vi "Dispose.vi"(8 "error in (no error)":errorcluster, 11 "ChangeNotifier in":refnum<class "ChangeNotifier.lvclass">) -> (0 "error out":errorcluster, 3 "ChangeNotifier out":refnum<class "ChangeNotifier.lvclass">)   [LabVIEW 2024, in "ChangeNotifier.lvclass"]
doc: "Destroy notifyChanges event."
uses:
  ChangeNotifier.lvclass
  ChangeNotifier.lvclass/ChangeNotifier.ctl
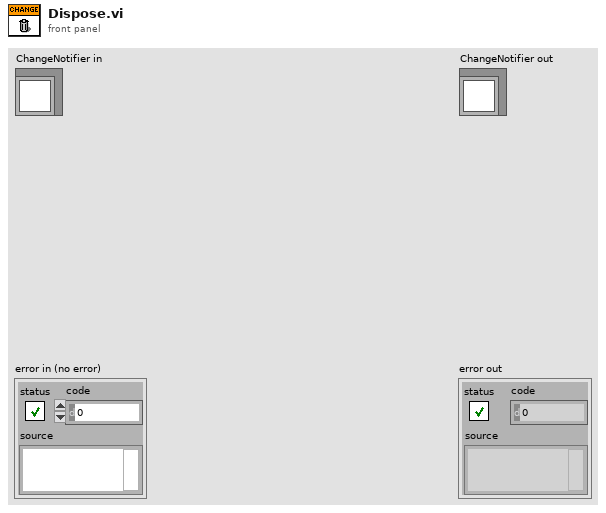
[diagram p1: front panel]
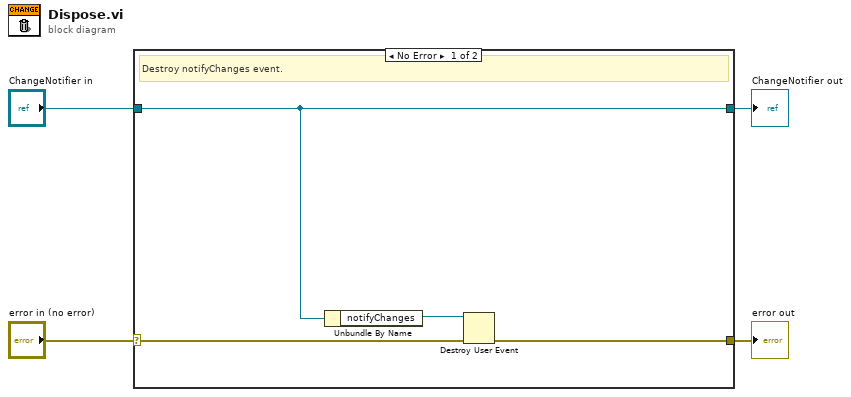
[diagram p0: block diagram]
diagram:
  n1 = case shown="No Error" "error in (no error)" {
    selector: "error in (no error)" -> [w6 w10]
    tunnel: [w5 w10] -> w3
    tunnel: [w7 w9] -> w1
    tunnel: "ChangeNotifier in" -> [w7 w9]
    frame No Error {
      # "Destroy notifyChanges event."
      n2 = Unbundle By Name(w7) -> ("notifyChanges"=w8:refnum<user-event>)
      n3 = Destroy User Event(user event=w8, error in=w6) -> (error out=w5:errorcluster)
    }
    frame Error {
    }
  }
  "error out" <- w3
  "ChangeNotifier out" <- w1
